vi "Add Structured Content.vi"(8 "error in":errorcluster, 10 "output info":T1(array[cluster]), 11 "response":string) -> (0 "error out":errorcluster, 3 "response out":string)   [LabVIEW 2020, in "MCP Server.lvlib"]
doc: "Adds structuredContent to a successful tools/call result.\n\nThe outputs of the tool are returned as one JSON object in the first text item of content. When the result is not marked with \"isError\": true, that object is copied into \"structuredContent\" of the result, without the outputs whose MCP type is picture (their images are separate image items of content). The text item stays as it is, so clients without structured output support see the same text as before.\n\nNo structuredContent is added when the result is an error result, when the text is not a JSON object, or when no output is left after the pictures are removed (a tool without outputs, or with pictures only).\n\nEvery other response is passed through."
uses:
  MCP Server.lvlib
  64511a0b-2976-4397-b7b7-7c5f1285976b.vi
  <vilib>/JDP Science/JSONtext/Next JSON Value.vi
  <vilib>/JDP Science/JSONtext/String Subset.vi
  <vilib>/JDP Science/JSONtext/Parsing/Advance past next JSON Value (inlined COPY).vi
  <vilib>/JDP Science/JSONtext/Parsing/Advance past whitespace.vi
  <vilib>/JDP Science/JSONtext/Parsing/Advance past String.vi
  <vilib>/JDP Science/JSONtext/Parsing/Advance past Number.vi
  <vilib>/JDP Science/JSONtext/Parsing/Advance past Line Ending.vi
  <vilib>/JDP Science/JSONtext/Parsing/Parse Full Path or Item Name.vi
  <vilib>/JDP Science/JSONtext/Parsing/Advance past Array.vi
  <vilib>/JDP Science/JSONtext/Parsing/Advance past Object.vi
  <vilib>/JDP Science/JSONtext/support/Error Cluster From Code.vi
  <vilib>/JDP Science/JSONtext/Offset/Find Item Locations by Path.vi
  <vilib>/JDP Science/JSONtext/JSON text to Variant.vi
  <vilib>/JDP Science/JSONtext/support/Format JSON Object.vi
  <vilib>/JDP Science/JSONtext/LVClass Serializer/JSONtext LVClass Serializer.lvclass
  <vilib>/JDP Science/JSONtext/JSONtext.lvlib
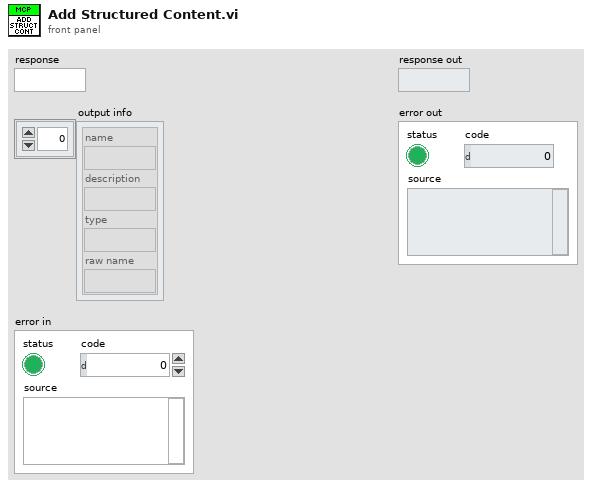
[diagram p1: front panel]
types:
  T1 = cluster{"name":string, "description":string, "type":string, "raw name":string}[]
  T2 = typedef "JSONtext.lvlib/JSON Value Type.ctl" = enum16{"Not a JSON Value", "JSON Object", "JSON Array", "String", "Number", "true", "false", "null"}
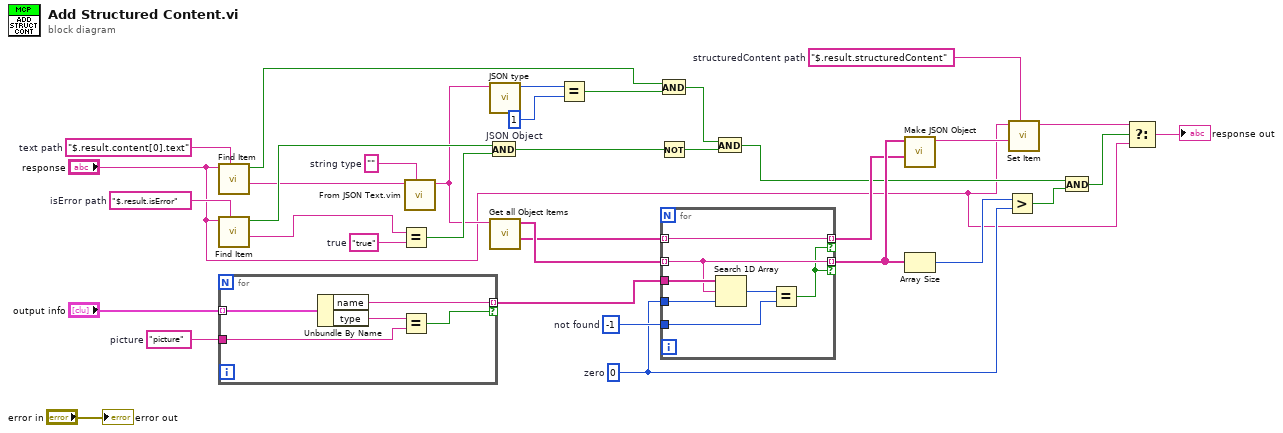
[diagram p0: block diagram]
diagram:
  w19 = -1  # not found
  w17 = 0  # zero
  w23 = "picture"  # picture
  w32 = "true"  # true
  w26 = u16 1  # JSON Object
  w28 = ""  # string type
  w13 = "$.result.structuredContent"  # structuredContent path
  w34 = "$.result.isError"  # isError path
  w35 = "$.result.content[0].text"  # text path
  n1 = call <vilib>:"Find Item.vi"("$Path or Item Name"=w35, "JSON"="response") -> ("<JSON>"=w29:string, "Found"=w11:bool)  [unwired: 6 in, 2 out]
  n2 = call <vilib>:"Find Item.vi"("$Path or Item Name"=w34, "JSON"="response") -> ("<JSON>"=w33:string, "Found"=w31:bool)  [unwired: 6 in, 2 out]
  n3 = for {
    tunnel: "output info" -> [w40] mode=indexing
    tunnel: w23 -> [w38]
    tunnel: [w36] -> w20 mode=indexing if=w37
    n4 = Unbundle By Name(w40) -> ("name"=w36:string, "type"=w39:string)
    n5 = Equal?(x=w39, y=w38) -> (x = y?=w37:bool)
  }
  n6 = Equal?(x=w33, y=w32) -> (x = y?=w30:bool)
  n7 = call "From JSON Text.vim"("Data Type and Default Value"=w28, "JSON"=w29) -> ("Data out"=w25:string)  [unwired: 8 in, 1 out]
  n8 = And(x=w31, y=w30) -> (x .and. y?=w12:bool)
  n9 = call <vilib>:"JSON type.vi"("JSON"=w25) -> ("JSON Value Type"=w27:T2)  [unwired: 9 in, 1 out]
  n10 = call <vilib>:"Get all Object Items.vi"("JSON"=w25) -> ("<JSON>"=w21:string[], "Item Names"=w22:string[])  [unwired: 7 in, 2 out]
  n11 = Equal?(x=w27, y=w26) -> (x = y?=w10:bool)
  n12 = And(x=w11, y=w10) -> (x .and. y?=w9:bool)
  n13 = Not(x=w12) -> (.not. x?=w8:bool)
  n14 = for {
    tunnel: w22 -> [w43] mode=indexing
    tunnel: w21 -> [w41] mode=indexing
    tunnel: w20 -> [w47]
    tunnel: w17 -> [w46]
    tunnel: w19 -> [w44]
    tunnel: [w43] -> w16 mode=indexing if=w42
    tunnel: [w41] -> w15 mode=indexing if=w42
    n15 = Search 1D Array(1D array=w47, element=w43, start index (0)=w46) -> (index of element=w45:i32)
    n16 = Equal?(x=w45, y=w44) -> (x = y?=w42:bool)
  }
  n17 = And(x=w9, y=w8) -> (x .and. y?=w7:bool)
  n18 = call <vilib>:"Make JSON Object.vi"("JSON Items"=w15, "Item Names"=w16) -> ("<JSON>"=w14:string)  [unwired: 8 in, 1 out]
  n19 = Array Size(array=w16) -> (size(s)=w18:i32)
  n20 = Greater?(x=w18, y=w17) -> (0:w6:bool)
  n21 = call <vilib>:"Set Item.vi"("$Path or Item Name"=w13, "JSON to Insert"=w14, "JSON"="response") -> ("<JSON>"=w5:string)  [unwired: 5 in, 2 out]
  n22 = And(x=w7, y=w6) -> (x .and. y?=w4:bool)
  n23 = Select(t=w5, s=w4, f="response") -> (s? t:f=→"response out":string)
  "error out" <- "error in"
